vi "CSM - Set TMO of Sync-Reply.vi"(8 "Error In":errorcluster caption="error in (no error)", 11 "TMO For Sync-Rep (ms) In":i32=5000) -> (0 "error out":errorcluster, 3 "TMO For Sync-Rep (ms) Out":i32=8000)   [LabVIEW 2017, in "Communicable State Machine.lvlib"]
doc: "Sets the global synchronous call timeout for the CSM program, in milliseconds. When the input is -2, the global timeout is not modified, and the return value is the current global timeout. When the input is any other positive value, the global timeout is modified to that value, and the new global timeout is returned.\n\n\n> [!NOTE] <b>CSM Synchronous Message Global Timeout</b>\n>\n> - When performing CSM inter-module communication or using the VI that sends synchronous messages, the default timeout is -2, which uses the globally configured timeout.\n> - The global timeout can be set to other positive values using the CSM - Set TMO of Sync-Reply VI to override the global setting.\n> - The global timeout only applies to synchronous calls. Asynchronous calls are unaffected.\n\n\nWhen calling a CSM Module/API, the default timeout is -2, in which case the globally configured timeout is used. If set to another positive value, that value is used as the timeout.\n\n-- <b>Controls</b> --\n- <b>TMO For Sync-Rep (ms) In</b>: Global timeout input. Using a value of -2 indicates no change to the global timeout. Other positive values indicate modifying the global timeout to that value.\n\n-- <b>Indicators</b> --\n- <b>TMO For Sync-Rep (ms) Out</b>: The current global timeout."
uses:
  Communicable State Machine.lvlib
  _Support/ChangeFlag/FlagInstance-Update CSMKVMap.vi
  _Support/ChangeFlag/ChangeFlag-Write.vi
  Utility/Random Change Flag.vi
  _Support/ChangeFlag/ChangeFlagDB.vi
  _Support/CSMKVMap/CSMKVMapDVR.vi
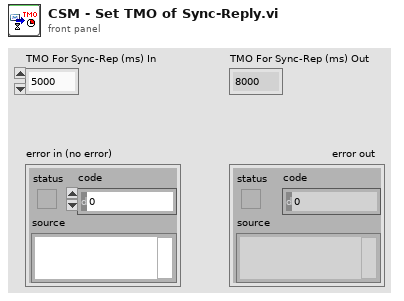
[diagram p1: front panel]
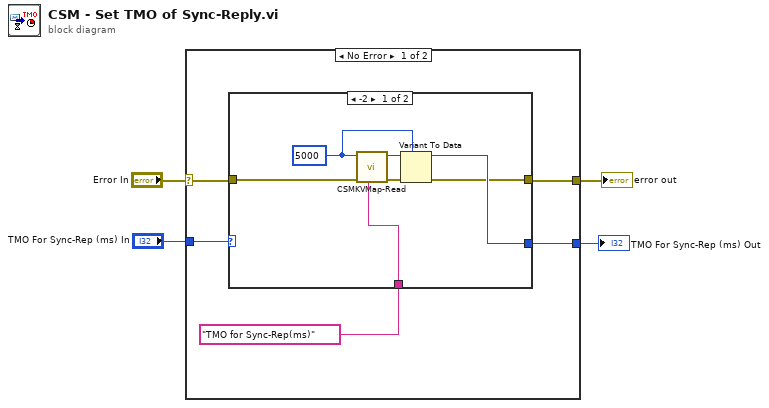
[diagram p0: block diagram]
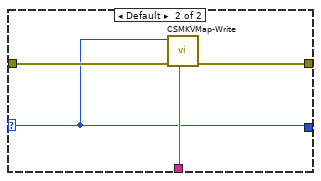
[diagram p2: hidden frame]
diagram:
  n1 = case shown="No Error" "Error In" {
    selector: "Error In" -> [w7 w21]
    tunnel: [w6 w21] -> w3
    tunnel: "TMO For Sync-Rep (ms) In" -> [w9 _]
    tunnel: [w8 _] -> w1
    frame No Error {
      n2 = case shown="-2" w9 {
        selector: w9 -> [_ w17]
        tunnel: [w13 w17] -> w8
        tunnel: [w12 w19] -> w6
        tunnel: w7 -> [w11 w20]
        tunnel: "TMO for Sync-Rep(ms)" ("name") -> [w10 w18]
        frame -2 {
          w14 = 5000 ("max queue size (-1, unlimited)")
          n3 = call "CSMKVMap-Read.vi"("name"=w10, "Error in"=w11, "default value (empty variant)"=w14) -> ("Error out"=w16:errorcluster, "value"=w15:variant)  [unwired: 5 in]
          n4 = Variant To Data(error in=w16, type=w14, Variant=w15) -> (data=w13:i32, error out=w12:errorcluster)
        }
        frame Default {
          n5 = call "CSMKVMap-Write.vi"("name"=w18, "Error in"=w20, "value"=w17) -> ("Error out"=w19:errorcluster)  [unwired: 6 in]
        }
      }
    }
    frame Error {
    }
  }
  "error out" <- w3
  "TMO For Sync-Rep (ms) Out" <- w1
